vi "Get Package Attributes.vi"(8 "error in":errorcluster, 10 "version":string, 11 "package name":string) -> (0 "error out":errorcluster, 1 "found?":bool, 2 "package attributes":T1={"Package Name"="", "Display name"="", "Version"="", "Display version"="", "Synopsis"="", "Description"="", "Maintainer"="", "Maintainer email address"="", "Category"="", "Homepage"="", "Release notes"="", "Depends"=[], "Recommends"=[], "Suggests"=[], "Conflicts"=[], "Provides"=[], "Replaces"=[], "Supplements"=[], "Enhances"=[], "Product"=FALSE, "User visible"=FALSE, "Installed size (KB)"=0, "Package filesize (bytes)"=0, "Architecture"="", "Agent"="file", "MD5Checksum"=""}, 3 "package name out":string)   [LabVIEW 2014, in "NIPM_API.lvlib"]
doc: "Returns the attributes for the specified version of a package\n\nINPUT(s)\n<B>Package name</B>: Specifies the package\n\n<B>Version</B>: Specifies the package version\n\nOUTPUT(s)\n<B>Package name out</B>: Outputs the package name\n\n<B>Package attributes</B>: Outputs the attributes for the specified version of the package\n\n<B>Found?</B>: Outputs whether this VI is able to find the specified version of the package in any of the registered feeds\n\nDETAILS:\nThis VI checks for package attribute data in both installed packages and packages in registered feeds."
uses:
  NIPM_API.lvlib
  _support/package attributes.ctl
panel:
  out "cmd standard output":string
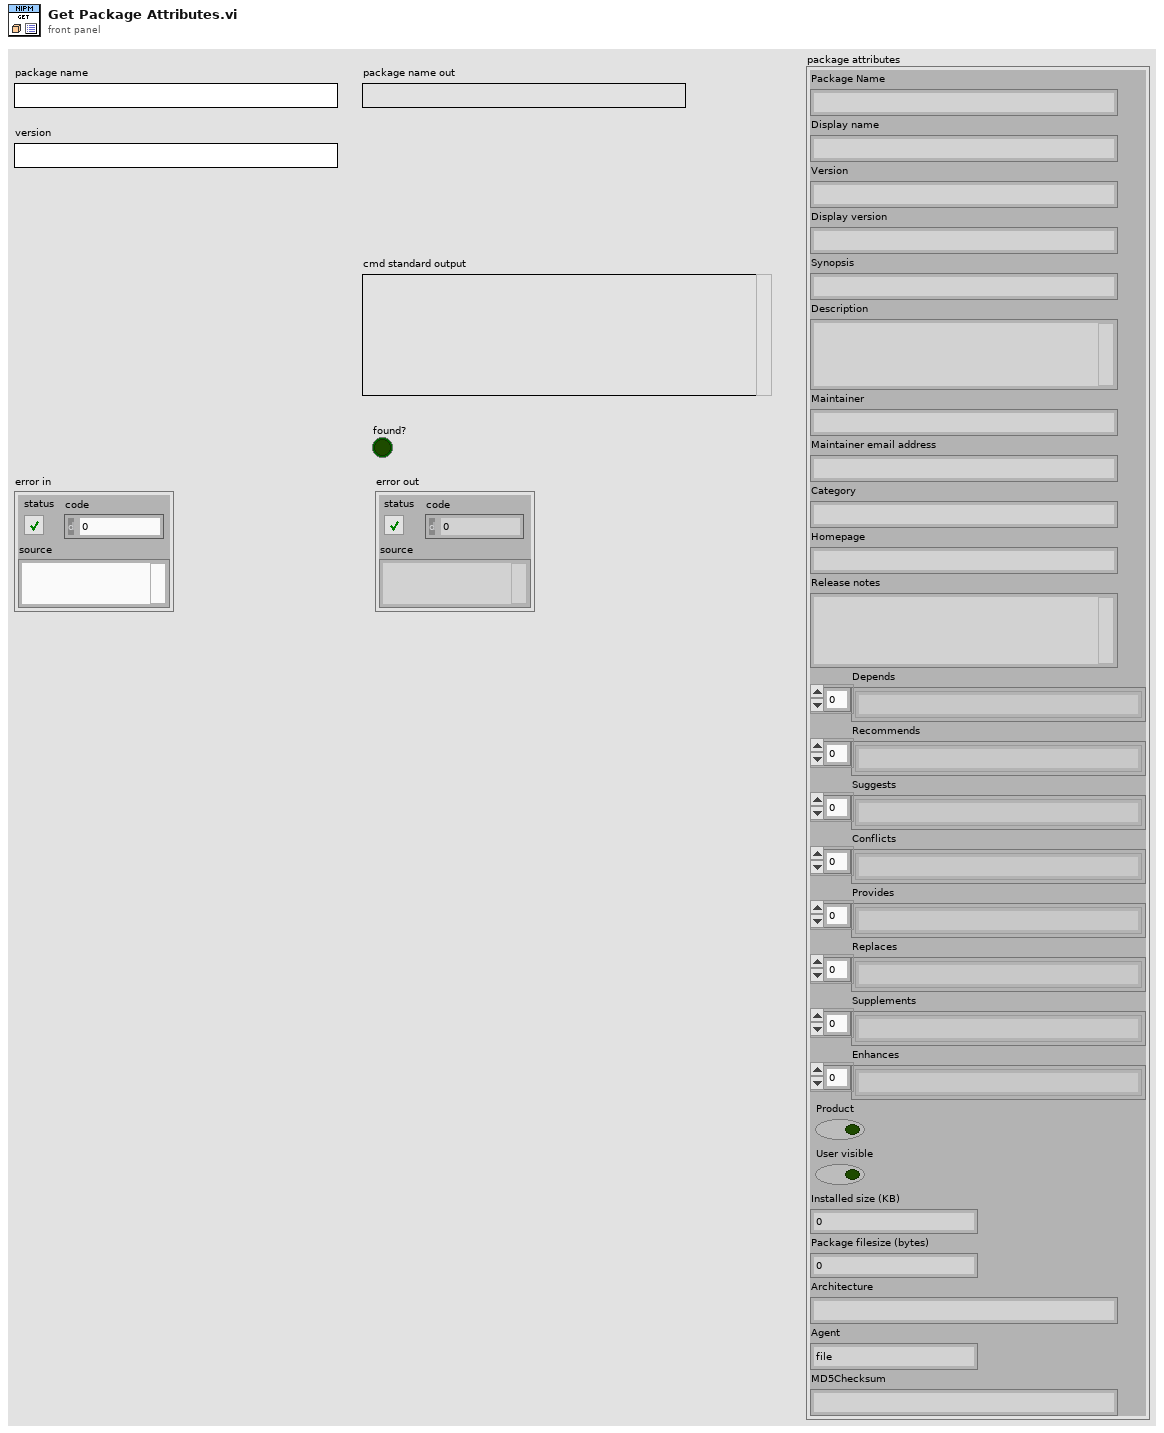
[diagram p1: front panel]
types:
  T1 = typedef "NIPM_API.lvlib/package attributes.ctl" = cluster{"Package Name":string, "Display name":string, "Version":string, "Display version":string, "Synopsis":string, "Description":string, "Maintainer":string, "Maintainer email address":string, "Category":string, "Homepage":string, "Release notes":string, "Depends":string[], "Recommends":string[], "Suggests":string[], "Conflicts":string[], "Provides":string[], "Replaces":string[], "Supplements":string[], "Enhances":string[], "Product":bool, "User visible":bool, "Installed size (KB)":u64, "Package filesize (bytes)":u64, "Architecture":string, "Agent":string, "MD5Checksum":string}
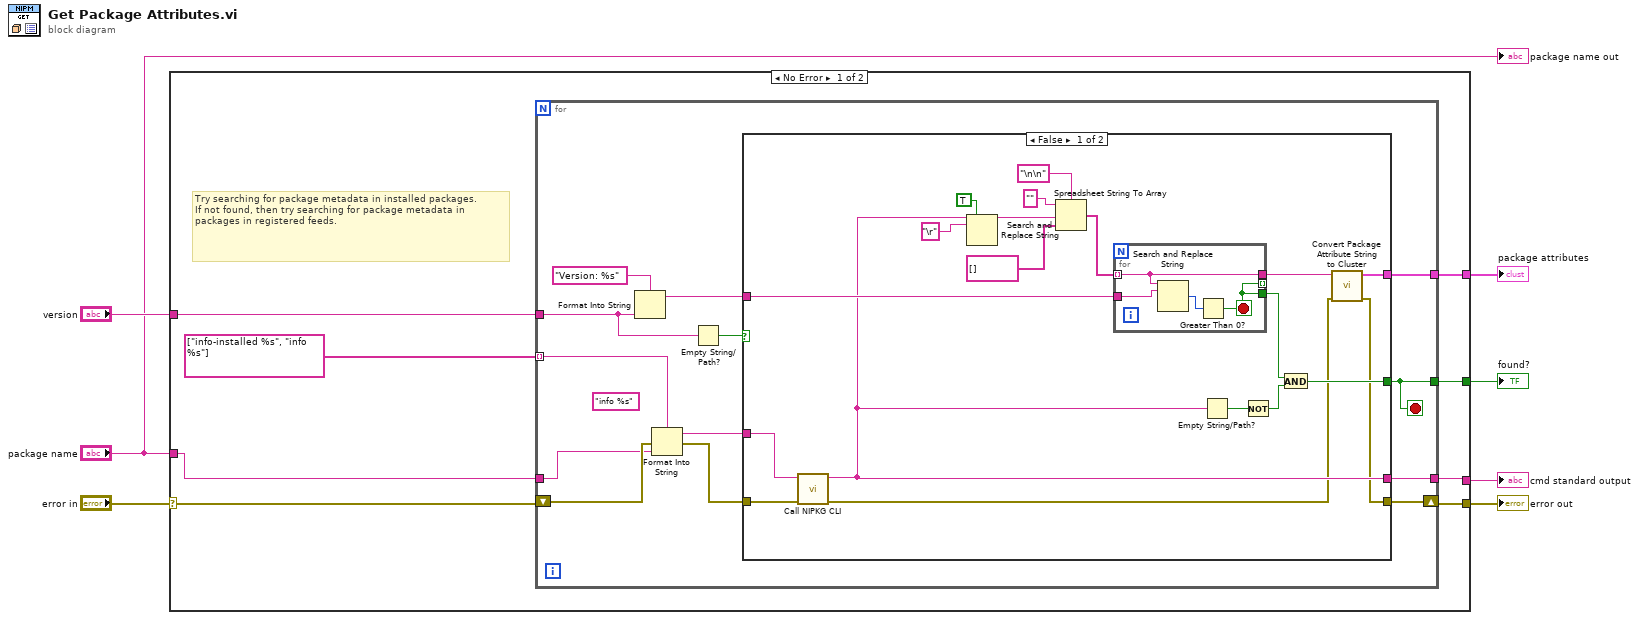
[diagram p0: block diagram]
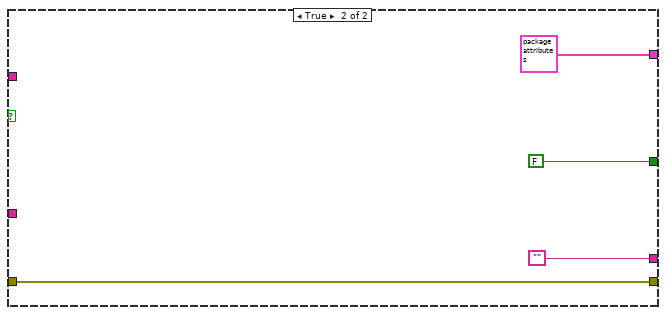
[diagram p2: hidden frame]
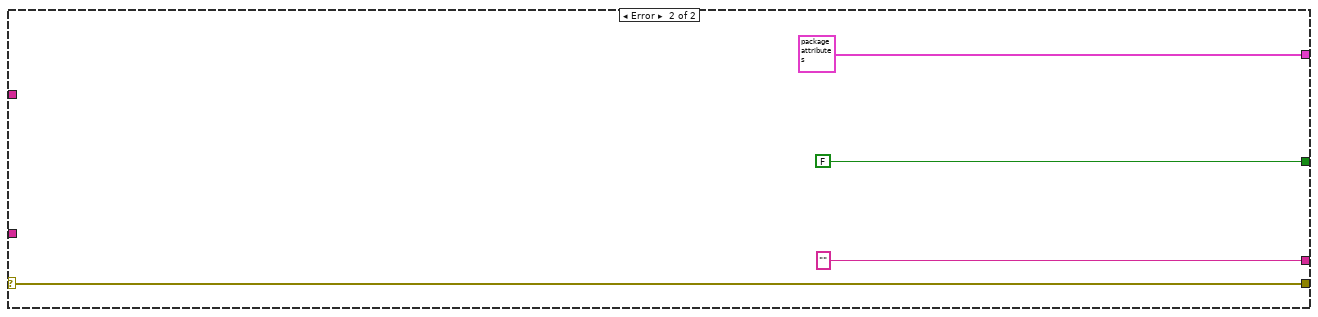
[diagram p3: hidden frame]
diagram:
  n1 = case shown="No Error" "error in" {
    selector: "error in" -> [w15 w59]
    tunnel: [w14 w59] -> w6
    tunnel: [w13 T1 {"Package Name"="", "Display name"="", "Version"="", "Display version"="", "Synopsis"="", "Description"="", "Maintainer"="", "Maintainer email address"="", "Category"="", "Homepage"="", "Release notes"="", "Depends"=[], "Recommends"=[], "Suggests"=[], "Conflicts"=[], "Provides"=[], "Replaces"=[], "Supplements"=[], "Enhances"=[], "Product"=FALSE, "User visible"=FALSE, "Installed size (KB)"=0, "Package filesize (bytes)"=0, "Architecture"="", "Agent"="file", "MD5Checksum"=""} ("package attributes")] -> w3
    tunnel: [w12 "" ("standard output")] -> w5
    tunnel: [w11 FALSE] -> w4
    tunnel: "version" -> [w10 _]
    tunnel: "package name" -> [w9 _]
    frame No Error {
      # "Try searching for package metadata in installed packages.\nIf not found, then try searching for package metadata in packages in registered feeds."
      n2 = for {
        tunnel: [w22] -> w13
        tunnel: [w16] -> w11
        tunnel: w10 -> [w19]
        shift-right: [w26] -> w14
        shift-left: w15 -> [w28]
        tunnel: string[] ["info-installed %s", "info %s"] -> [w17] mode=indexing
        tunnel: w9 -> [w18]
        tunnel: [w21] -> w12
        stop <- w16 stop-if-true
        (unwired) "info %s" ("format string")
        n3 = Format Into String(format string="Version: %s", w19) -> (resulting string=w23:string)  [unwired: 2 in, 1 out]
        n4 = Format Into String(format string=w17, error in=w28, w18) -> (resulting string=w25:string, error out=w27:errorcluster)  [unwired: 1 in]
        n5 = Empty String/Path?(string/path=w19) -> (empty?=w20:bool)
        n6 = case shown="False" w20 {
          tunnel: w27 -> [w34 w54]
          tunnel: [w29 w54] -> w26
          tunnel: w25 -> [w35 _]
          tunnel: w23 -> [w40 _]
          tunnel: [w31 T1 {"Package Name"="", "Display name"="", "Version"="", "Display version"="", "Synopsis"="", "Description"="", "Maintainer"="", "Maintainer email address"="", "Category"="", "Homepage"="", "Release notes"="", "Depends"=[], "Recommends"=[], "Suggests"=[], "Conflicts"=[], "Provides"=[], "Replaces"=[], "Supplements"=[], "Enhances"=[], "Product"=FALSE, "User visible"=FALSE, "Installed size (KB)"=0, "Package filesize (bytes)"=0, "Architecture"="", "Agent"="file", "MD5Checksum"=""} ("package attributes")] -> w22
          tunnel: [w33 ""] -> w21
          tunnel: [w39 FALSE] -> w16
          frame False {
            n7 = call "Call NIPKG CLI.vi"("error in (no error)"=w34, "command"=w35) -> ("error out"=w30:errorcluster, "command line standard output"=w33:string)  [unwired: 8 in]
            n8 = Search and Replace String(replace all?=TRUE ("replace all? (F)"), input string=w33, search string="\r") -> (result string=w45:string)  [unwired: 5 in, 3 out]
            n9 = Spreadsheet String To Array(delimiter (Tab)="\n\n", format string="", spreadsheet string=w45, array type (2D Dbl)=string[] []) -> (array=w41:string[])
            n10 = for {
              tunnel: w41 -> [w49] mode=indexing
              tunnel: w40 -> [w50]
              tunnel: [w49] -> w32 if=w51
              tunnel: [w51] -> _ mode=indexing
              tunnel: [w51] -> w36
              stop <- w51 stop-if-true
              n11 = Search and Replace String(input string=w49, search string=w50) -> (number of replacements=w48:i32)  [unwired: 6 in, 3 out]
              n12 = Greater Than 0?(x=w48) -> (x > 0?=w51:bool)
            }
            n13 = Empty String/Path?(string/path=w33) -> (empty?=w38:bool)
            n14 = Not(x=w38) -> (.not. x?=w37:bool)
            n15 = And(x=w36, y=w37) -> (x .and. y?=w39:bool)
            n16 = call "Convert Package Attribute String to Cluster.vi"("error in (no error)"=w30, "package attributes string"=w32) -> ("error out"=w29:errorcluster, "package attributes"=w31:T1)  [unwired: 8 in]
          }
          frame True {
          }
        }
      }
    }
    frame Error {
    }
  }
  "error out" <- w6
  "cmd standard output" <- w5
  "found?" <- w4
  "package attributes" <- w3
  "package name out" <- "package name"
